vi "ProgramStatus.vi"(0 "Universal Robot.lvclass in":refnum<class "Universal Robot.lvclass">, 5 "error in (no error)":errorcluster) -> (14 "Universal Robot.lvclass out":refnum<class "Universal Robot.lvclass">, 15 "Program Status":T1, 19 "error out":errorcluster)   [LabVIEW 2019, in "Universal Robot.lvclass"]
uses:
  Universal Robot.lvclass
  ProgramStatus.ctl
  ProgramState.ctl
  Universal Robot.lvclass/Universal Robot.ctl
  Client Interfaces/Dashboard Server/Dashboard Server.lvclass
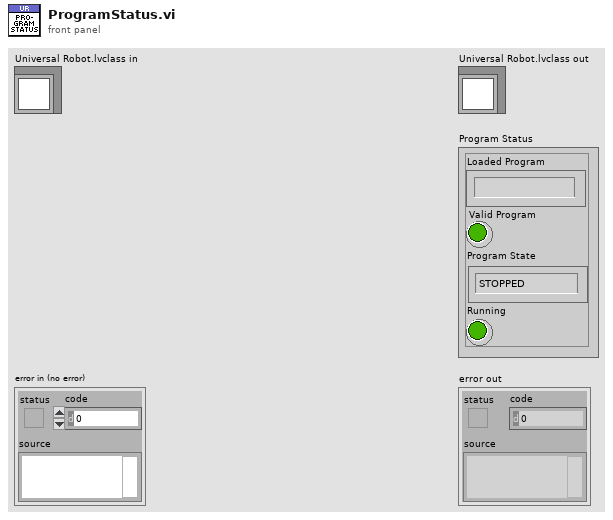
[diagram p1: front panel]
types:
  T1 = typedef "Universal Robot.lvclass/ProgramStatus.ctl" = cluster{"Loaded Program":string, "Valid Program":bool, "Program State":T2, "Running":bool}
  T2 = typedef "Universal Robot.lvclass/ProgramState.ctl" = enum16{"STOPPED", "PLAYING", "PAUSE"}
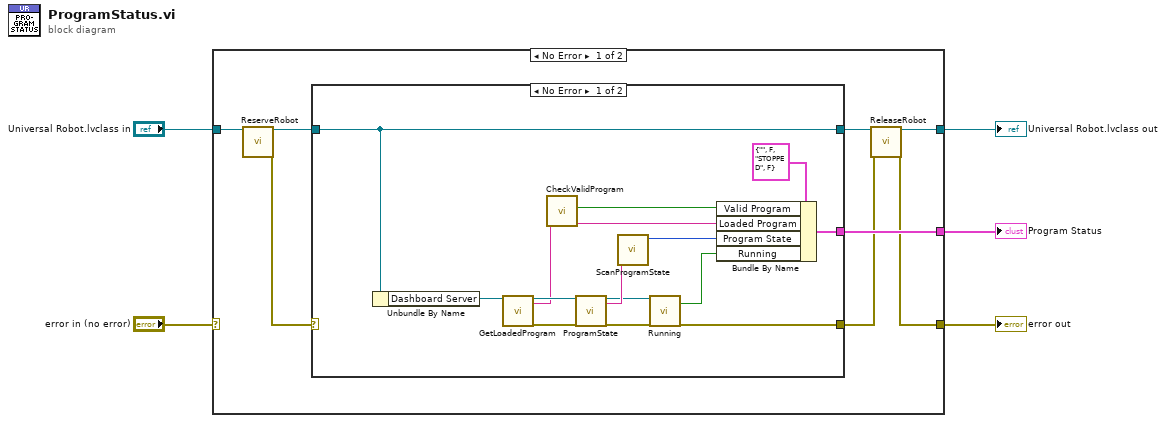
[diagram p0: block diagram]
diagram:
  n1 = case shown="No Error" "error in (no error)" {
    selector: "error in (no error)" -> [_ w32]
    tunnel: [w6 w32] -> w4
    tunnel: "Universal Robot.lvclass in" -> [w12 w31]
    tunnel: [w8 w31] -> w2
    tunnel: [w13 _] -> w1
    frame No Error {
      n2 = call "ReserveRobot.vi"("Universal Robot.lvclass in"=w12) -> ("Universal Robot.lvclass out"=w11:refnum<class "Universal Robot.lvclass">, "error out"=w10:errorcluster)  [unwired: 17 in]
      n3 = case shown="No Error" w10 {
        selector: w10 -> [_ w30]
        tunnel: [w28 _] -> w13
        tunnel: w11 -> [w15 w29]
        tunnel: [w15 w29] -> w9
        tunnel: [w14 w30] -> w7
        frame No Error {
          n4 = Unbundle By Name(w15) -> ("Dashboard Server"=w26:refnum<class "Dashboard Server.lvclass">)
          n5 = call-dynamic "GetLoadedProgram.vi"("DashboardServer in"=w26) -> ("DashboardServer out"=w25:refnum<class "Dashboard Server.lvclass">, "loadedProgram"=w18:string, "error out"=w24:errorcluster)  [unwired: 16 in]
          n6 = call "CheckValidProgram.vi"("loadedProgram in"=w18) -> ("loadedProgram out"=w17:string, "valid?"=w16:bool)  [unwired: 9 in]
          n7 = call-dynamic "ProgramState.vi"("DashboardServer in"=w25, "error in (no error)"=w24) -> ("DashboardServer out"=w21:refnum<class "Dashboard Server.lvclass">, "programState"=w23:string, "error out"=w20:errorcluster)  [unwired: 15 in]
          n8 = call "ScanProgramState.vi"("programState in"=w23) -> ("programState out"=w22:T2)  [unwired: 10 in]
          n9 = call-dynamic "Running.vi"("DashboardServer in"=w21, "error in (no error)"=w20) -> ("running"=w19:bool, "error out"=w14:errorcluster)  [unwired: 15 in, 1 out]
          n10 = Bundle By Name(cluster=T1 {"Loaded Program"="", "Valid Program"=FALSE, "Program State"=enum."STOPPED", "Running"=FALSE} ("Program Status"), "Valid Program"=w16, "Loaded Program"=w17, "Program State"=w22, "Running"=w19) -> (w28:T1)
        }
        frame Error {
        }
      }
      n11 = call "ReleaseRobot.vi"("Universal Robot.lvclass in"=w9, "error in (no error)"=w7) -> ("Universal Robot.lvclass out"=w8:refnum<class "Universal Robot.lvclass">, "error out"=w6:errorcluster)  [unwired: 16 in]
    }
    frame Error {
    }
  }
  "error out" <- w4
  "Universal Robot.lvclass out" <- w2
  "Program Status" <- w1
